vi "MQTT Properties - Get.vi"(0 "MQTT Properties":cluster{"Property":u8, "Value":string}[](array[cluster]), 7 "MQTT Property Type":T1=17 items=["Payload Format Indicator"=1, "Message Expiry Interval"=2, "Content Type"=3, "Response Topic"=8, "Correlation Data"=9, "Subscription Identifier"=11, "Session Expiry Interval"=17, "Assigned Client Identifier"=18, "Server Keep Alive"=19, "Authentication Method"=21, "Authentication Data"=22, "Request Problem Information"=23, "Will Delay Interval"=24, "Request Response Information"=25, "Response Information"=26, "Server Reference"=28, "Reason String"=31, "Receive Maximum"=33, "Topic Alias Maximum"=34, "Topic Alias"=35, "Maximum QoS"=36, "Retain Available"=37, "User Property"=38, "Maximum Packet Size"=39, "Wildcard Subscription Available"=40, "Subscription Identifier Available"=41, "Shared Subscription Available"=42]) -> (4 "MQTT Properties out":cluster{"Property":u8, "Value":string}[](array[cluster]), 6 "Found":bool, 8 "Value":string)   [LabVIEW 2019, in "KoRE-MQTT.lvlib"]
doc: "Copyright (c) 2025 KoRElibs.com\nSPDX-License-Identifier: EUPL-1.2\n\nThis VI is licensed under the European Union Public License (EUPL) Version 1.2. You may use this VI unmodified in proprietary works. If you distribute a modified version of this file, the modified file must be released under the EUPL-1.2. Full license: https://joinup.ec.europa.eu/asset/eupl/eupl/1.2/"
uses:
  KoRE-MQTT.lvlib
  TypeDefs/MQTT Property Type.ctl
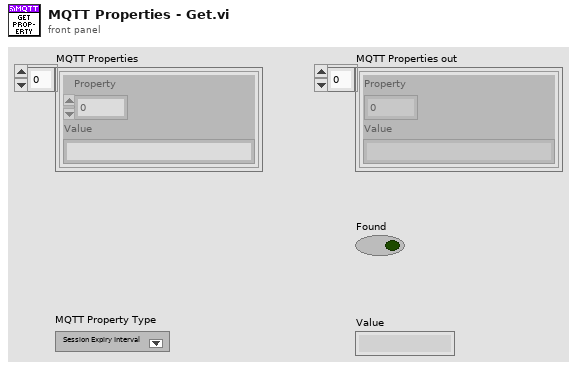
[diagram p1: front panel]
types:
  T1 = typedef "KoRE-MQTT.lvlib/MQTT Property Type.ctl" = u8
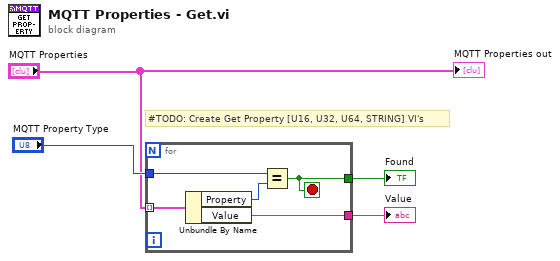
[diagram p0: block diagram]
diagram:
  # "#TODO: Create Get Property [U16, U32, U64, STRING] VI's"
  n1 = for {
    tunnel: "MQTT Properties" -> [w9] mode=indexing
    tunnel: "MQTT Property Type" -> [w7]
    tunnel: [w6] -> w4
    tunnel: [w5] -> w3
    stop <- w6 stop-if-true
    n2 = Unbundle By Name(w9) -> ("Property"=w8:u8, "Value"=w5:string)
    n3 = Equal?(x=w7, y=w8) -> (x = y?=w6:bool)
  }
  "Found" <- w4
  "Value" <- w3
  "MQTT Properties out" <- "MQTT Properties"
